vi "Write OD Vars.vi"(8 "error in (no error)":errorcluster, 10 "OD Vars":T1[](array[typedef]) {"CANOpen Types" items=["bool"=1, "i8"=2, "i16"=3, "i32"=4, "u8"=5, "u16"=6, "u32"=7, "f32"=8, "visible str"=9, "octet str"=10, "f64"=17, "i64"=21, "u64"=27]; "OD Index"."SubIndex" format="%.0x"; "OD Index"."Index" format="%.0x"}, 11 "OD Batch in":refnum<class "OD Batch.lvclass">) -> (0 "error out":errorcluster, 3 "OD Batch out":refnum<class "OD Batch.lvclass">)   [LabVIEW 2023, in "xnet_canopen.lvlib" / "OD Batch.lvclass"]
uses:
  OD Batch.lvclass
  OD Batch.lvclass/OD Batch.ctl
  typedef/od index.ctl
  xnet_canopen.lvlib
  typedef/canopen types.ctl
  typedef/od entry.ctl
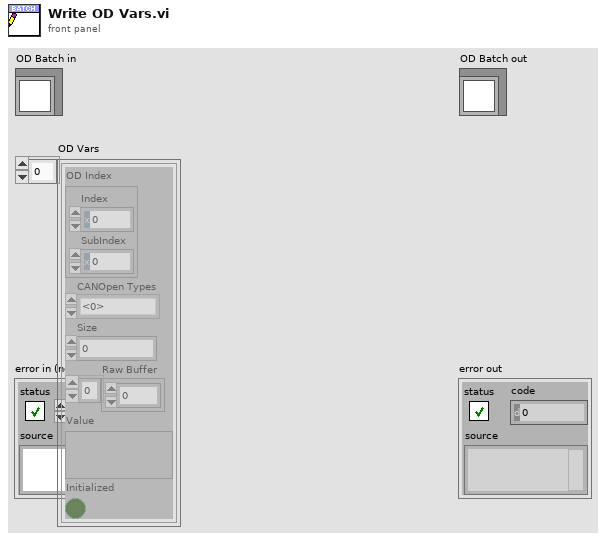
[diagram p1: front panel]
types:
  T1 = typedef "xnet_canopen.lvlib/od entry.ctl" = cluster{"OD Index":T2, "CANOpen Types":T3, "Size":u32, "Raw Buffer":u8[], "Value":variant, "Initialized":bool}
  T2 = typedef "xnet_canopen.lvlib/od index.ctl" = cluster{"Index":u16, "SubIndex":u8}
  T3 = typedef "xnet_canopen.lvlib/canopen types.ctl" = u32
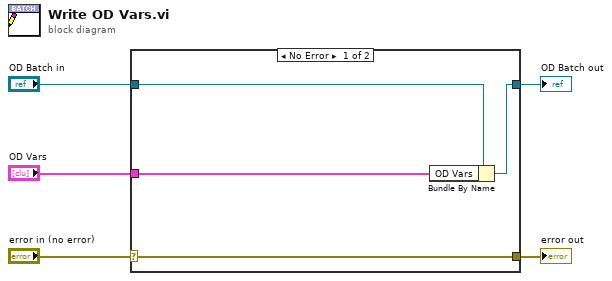
[diagram p0: block diagram]
diagram:
  n1 = case shown="No Error" "error in (no error)" {
    selector: "error in (no error)" -> [w9 w10]
    tunnel: [w9 w10] -> w4
    tunnel: [w7 w11] -> w2
    tunnel: "OD Batch in" -> [w8 w11]
    tunnel: "OD Vars" -> [w6 _]
    frame No Error {
      n2 = Bundle By Name(cluster=w8, "OD Vars"=w6) -> (w7:refnum<class "OD Batch.lvclass">)
    }
    frame Error {
    }
  }
  "error out" <- w4
  "OD Batch out" <- w2
